vi "Add Child Items to Tree.vi"(8 "error in (no error)":errorcluster, 10 "Polymorphic VI Type in":refnum<class "Polymorphic VI Type.lvclass">, 11 "Tree Ref in":refnum<vi>) -> (0 "error out":errorcluster, 2 "Polymorphic VI Type out":refnum<class "Polymorphic VI Type.lvclass">, 3 "Tree Ref out":refnum<vi>)   [LabVIEW 2020, in "Peek Window.lvlib" / "Polymorphic VI Type.lvclass"]
uses:
  Polymorphic VI Type.lvclass
  C:/Users/mjacobso/Desktop/SCM/VI-Peek/source/Peek Window/VI Types/Standard VI Type/Standard VI Type.lvclass
  Polymorphic VI Type.lvclass/Polymorphic VI Type.ctl
  Standard VI Type/Standard VI Type.lvclass/Standard VI Type.ctl
  Symbols Enum.ctl
  Standard VI Type/Read Full Qualified Name.vi
  Implementation VI Type/Implementation VI Type.lvclass
  Peek Window.lvlib
  Standard VI Type/Standard VI Type.lvclass
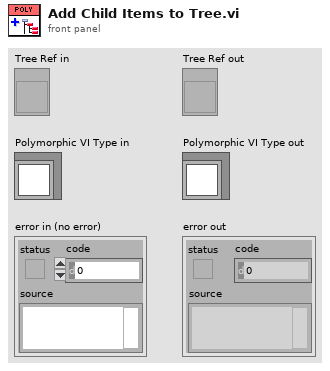
[diagram p1: front panel]
types:
  T1 = map{string, refnum<class "Implementation VI Type.lvclass">}
  T2 = cluster{"VIPath":path, "Menu Name":string, "Selector Name":string}[]
  T3 = typedef "Peek Window.lvlib/Symbols Enum.ctl" = enum16{"<Blank>", "Implementation Mark", "Standard VI", "Dynamic Dispatch VI", "Malleable VI", "Polymorphic VI", "Missing VI", "Express VI"}
  T4 = typedef "Peek Window.lvlib/Polymorphic VI Type.lvclass/Selected Item Enum.ctl" = enum16{"Polymorphic", "Instance"}
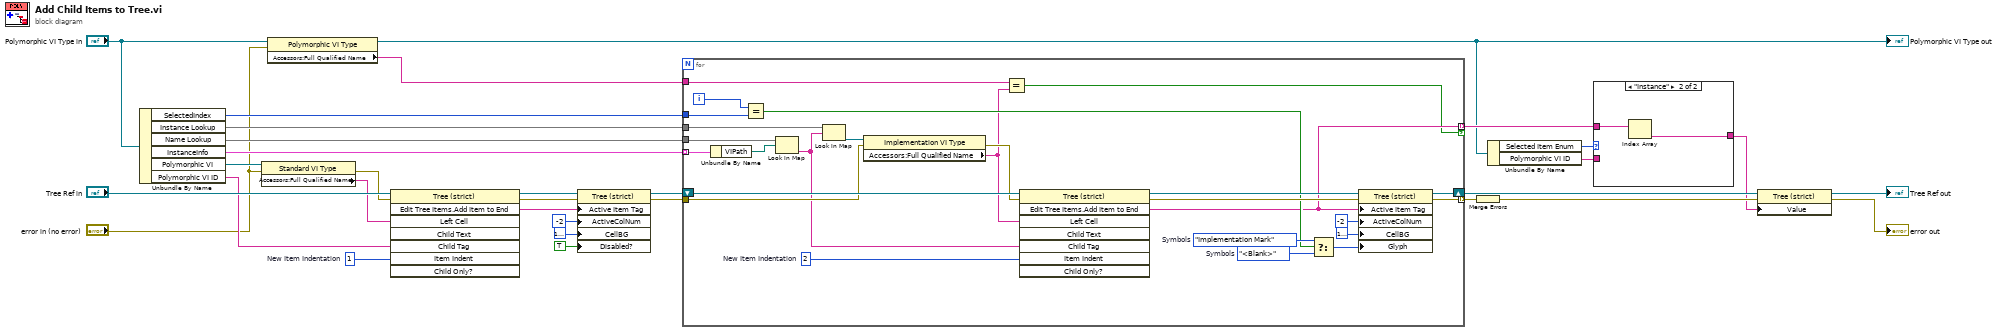
[diagram p0: block diagram]
diagram:
  w29 = 1  # New Item Indentation
  n1 = Unbundle By Name("Polymorphic VI Type in") -> ("SelectedIndex"=w14:i32, "Instance Lookup"=w13:T1, "Name Lookup"=w17:map{path, string}, "InstanceInfo"=w20:T2, "Polymorphic VI"=w31:refnum<class "Standard VI Type.lvclass">, "Polymorphic VI ID"=w16:string)
  n2 = property class="Standard VI Type"(reference=w31, error in="error in (no error)") -> (error out=w23:errorcluster, "Accessors:Full Qualified Name"=w15:string)  [unwired: 1 out]
  n3 = property class="Polymorphic VI Type"(reference="Polymorphic VI Type in", error in="error in (no error)") -> (reference out=w4:refnum<class "Polymorphic VI Type.lvclass">, "Accessors:Full Qualified Name"=w2:string)  [unwired: 1 out]
  "Polymorphic VI Type out" <- w4
  n4 = invoke class="Tree (strict)" method="Edit Tree Items.Add Item to End"(reference="Tree Ref in", error in=w23, "Left Cell"=w15, "Child Tag"=w16, "Item Indent"=w29) -> (reference out=w26:refnum<vi>, error out=w24:errorcluster, "Edit Tree Items:Add Item to End"=w25:string)  [unwired: 3 in, 5 out]
  n5 = property class="Tree (strict)"(reference=w26, error in=w24, "Active Item Tag"=w25, "ActiveColNum"=-2, "CellBG"=u32 16777238, "Disabled?"=TRUE ("Active Item:Disabled?")) -> (reference out=w21:refnum<vi>, error out=w22:errorcluster)
  n6 = for {
    tunnel: w22 -> [w38]
    shift-right: [w51] -> w11
    shift-left: w21 -> [w52]
    tunnel: w20 -> [w49] mode=indexing
    tunnel: [w50] -> w19 mode=indexing
    tunnel: w14 -> [w47]
    tunnel: w17 -> [w43]
    tunnel: w13 -> [w41]
    tunnel: [w35] -> w8 mode=indexing if=w32
    tunnel: w2 -> [w34]
    i -> [w48]
    w45 = Symbols_Enum."<Blank>"  # Symbols
    w46 = Symbols_Enum."Implementation Mark"  # Symbols
    w53 = 2  # New Item Indentation
    n7 = Unbundle By Name(w49) -> ("VIPath"=w42:path)
    n8 = Equal?(x=w48, y=w47) -> (x = y?=w36:bool)
    n9 = Look In Map(map=w43, key=w42) -> (value=w37:string)  [unwired: 1 in, 1 out]
    n10 = Look In Map(map=w41, key=w37) -> (value=w40:refnum<class "Implementation VI Type.lvclass">)  [unwired: 1 in, 1 out]
    n11 = property class="Implementation VI Type"(reference=w40, error in=w38) -> (error out=w39:errorcluster, "Accessors:Full Qualified Name"=w33:string)  [unwired: 1 out]
    n12 = Equal?(x=w34, y=w33) -> (x = y?=w32:bool)
    n13 = invoke class="Tree (strict)" method="Edit Tree Items.Add Item to End"(reference=w52, error in=w39, "Left Cell"=w33, "Child Tag"=w37, "Item Indent"=w53) -> (reference out=w56:refnum<vi>, error out=w57:errorcluster, "Edit Tree Items:Add Item to End"=w35:string)  [unwired: 3 in, 5 out]
    n14 = Select(t=w46, s=w36, f=w45) -> (s? t:f=w44:T3)
    n15 = property class="Tree (strict)"(reference=w56, error in=w57, "Active Item Tag"=w35, "ActiveColNum"=-2, "CellBG"=u32 16777238, "Glyph"=w44) -> (reference out=w51:refnum<vi>, error out=w50:errorcluster)
  }
  n16 = Merge Errors(w19) -> (w18:errorcluster)
  n17 = Unbundle By Name(w4) -> ("Selected Item Enum"=w7:T4, "Polymorphic VI ID"=w5:string)
  n18 = case shown="\"Instance\"" w7 {
    tunnel: w8 -> [_ w60]
    tunnel: [w58 w59] -> w6
    tunnel: w5 -> [w58 _]
    frame "Polymorphic" {
    }
    frame "Instance" {
      n19 = Index Array(array=w60) -> (element=w59:string)  [unwired: 1 in]
    }
  }
  n20 = property class="Tree (strict)"(reference=w11, error in=w18, "Value"=w6) -> (reference out=→"Tree Ref out":refnum<vi>, error out=→"error out":errorcluster)
